vi "K_S30 Terminal-CN.vi"(8 "error in":errorcluster, 10 "request":u8[](array[numeric]), 11 "VISA resource":refnum<visa-resource-name>="COM2") -> (0 "error out":errorcluster, 2 "response":u8[](array[numeric]))   [LabVIEW 2022 SP3]
panel:
  out "msg and CRC":u8[](array[numeric])
  out "delited":u8[](array[numeric])
  # "Terminal for KELLER Transmitters Series3x \nV1.0, b.v.\n\nConfigure ComPort: use K_S30 OpenComPort --> Global Variable\n\nsend a message with CRC16 checksum, receive the reponse\ncheck CRC16, and exceptions\n\nerrors:\n0: no error\n1,2,3,32: exceptions thrown by the device: see comm. protocol\n100: broadcast\n-2: wrong echo from the RS485 converter\n-4: timeout\n-5: CRC16 wrong\nothers thrown by VISA"
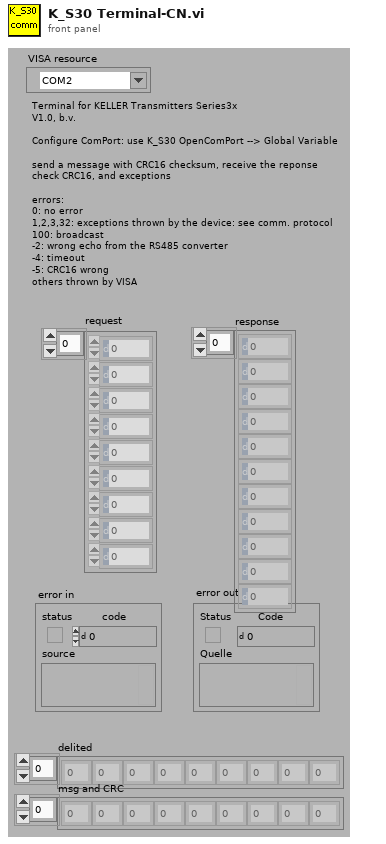
[diagram p1: front panel]
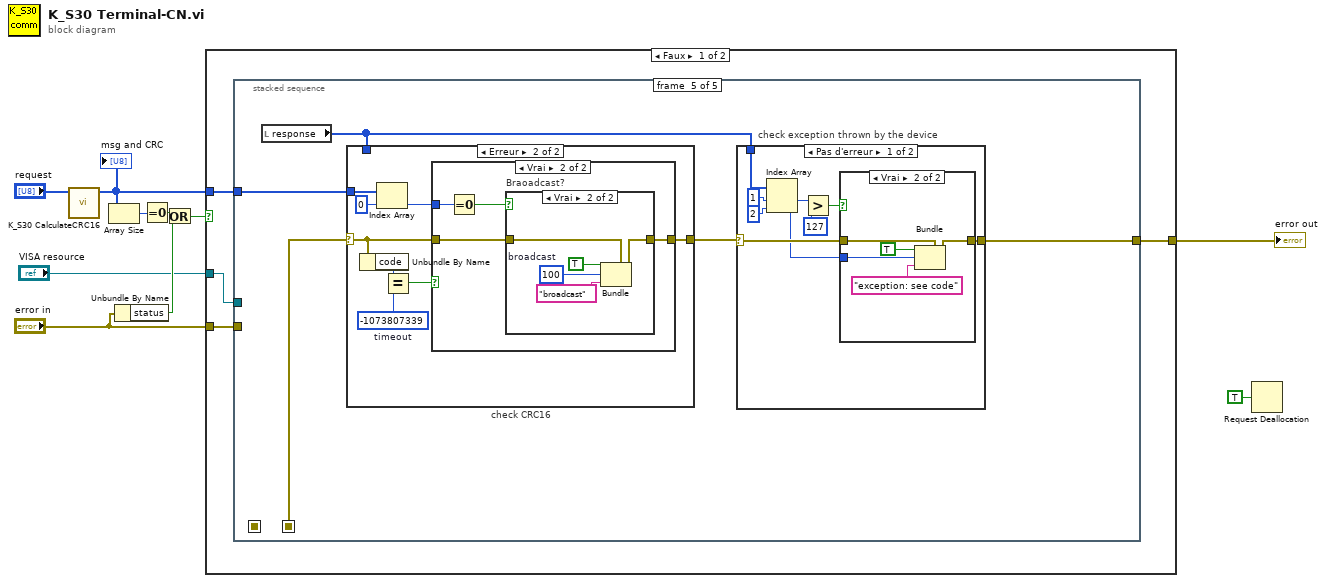
[diagram p0: block diagram]
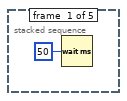
[diagram p2: hidden frame]
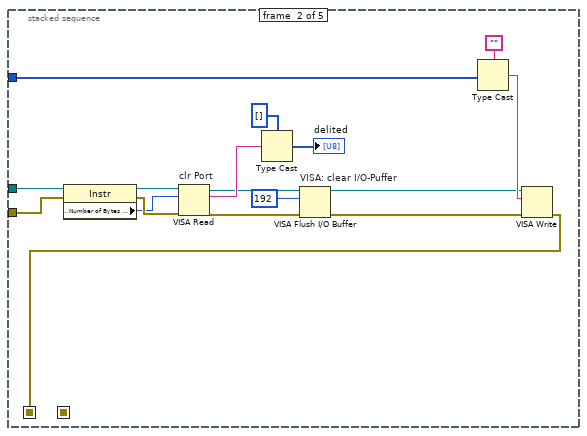
[diagram p3: hidden frame]
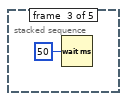
[diagram p4: hidden frame]
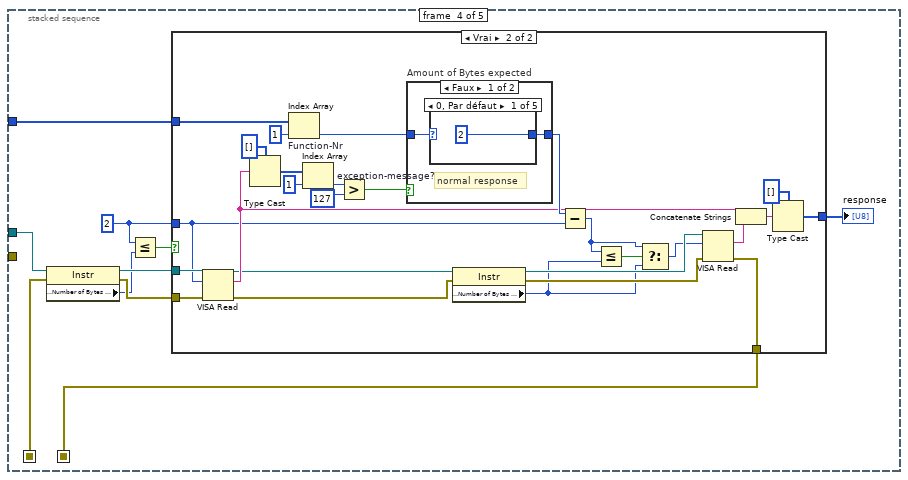
[diagram p5: hidden frame]
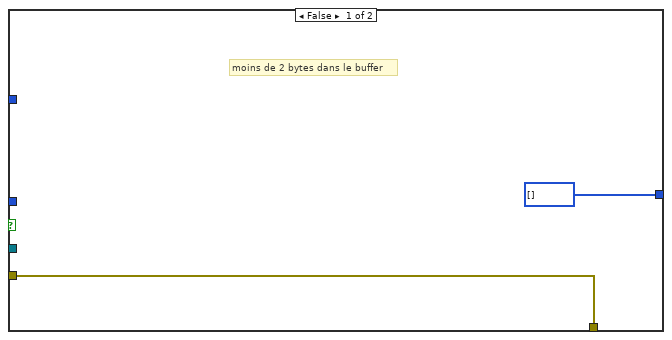
[diagram p6: hidden frame]
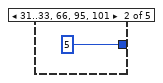
[diagram p7: hidden frame]
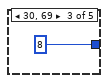
[diagram p8: hidden frame]
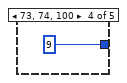
[diagram p9: hidden frame]
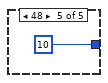
[diagram p10: hidden frame]
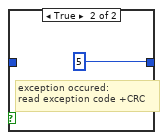
[diagram p11: hidden frame]
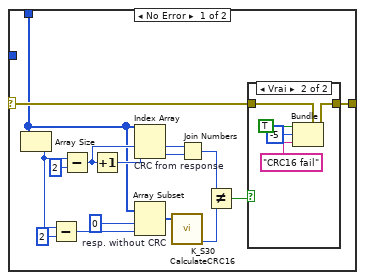
[diagram p14: hidden frame]
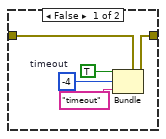
[diagram p17: hidden frame]
diagram:
  n1 = call "K_S30 CalculateCRC16.vi"("msg without CRC"="request") -> ("msg and CRC"=w4:u8[])  [unwired: 3 in, 3 out]
  "msg and CRC" <- w4
  n2 = Array Size(array=w4) -> (size(s)=w5:i32)
  n3 = Unbundle By Name("error in") -> ("status"=w7:bool)
  n4 = Equal To 0?(x=w5) -> (x = 0?=w8:bool)
  n5 = Or(x=w8, y=w7) -> (x .or. y?=w6:bool)
  n6 = case shown="Faux" w6 {
    tunnel: "VISA resource" -> [w14 _]
    tunnel: "error in" -> [w13 w147]
    tunnel: w4 -> [w12 _]
    tunnel: [w11 w147] -> w3
    frame False {
      n7 = stacked-sequence {
        seq-local: [_ w16 _ _ _] -> [_ _ _ w39 _]
        seq-local: [_ _ _ w41 _] -> [_ _ _ _ w82]
        tunnel: w14 -> [_ w28 _ w40 _]
        tunnel: w13 -> [_ w27 _ _ _]
        tunnel: w12 -> [_ w17 _ w43 w81]
        tunnel: [_ _ _ _ w83] -> w11
        frame #0 {
          n8 = Wait (ms)(milliseconds to wait=u32 50 ("ms Wartezeit")) -> ()  [unwired: 1 out]
        }
        frame #1 {
          n9 = property class="Instr"(reference=w28, error in=w27) -> (reference out=w32:refnum<visa-resource-name>, error out=w31:errorcluster, "Serial Settings:Number of Bytes at Serial Port"=w30:u32)
          n10 = VISA Read "clr Port"(VISA resource name=w32, byte count=w30, error in (no error)=w31) -> (VISA resource name out=w23:refnum<visa-resource-name>, read buffer=w26:string, error out=w24:errorcluster)  [unwired: 1 out]
          n11 = Type Cast(type=u8[] [], x=w26) -> (*(type *) &x=→"delited":u8[])
          n12 = VISA Flush I/O Buffer "VISA: clear I/O-Puffer"(VISA resource name=w23, mask (16)=u16 192 ("Maskieren (16)"), error in (no error)=w24) -> (VISA resource name out=w19:refnum<visa-resource-name>, error out=w18:errorcluster)
          n13 = Type Cast(type="", x=w17) -> (*(type *) &x=w20:string)
          n14 = VISA Write(VISA resource name=w19, write buffer=w20, error in (no error)=w18) -> (error out=w16:errorcluster)  [unwired: 2 out]
        }
        frame #2 {
          n15 = Wait (ms)(milliseconds to wait=u32 50 ("ms Wartezeit")) -> ()  [unwired: 1 out]
        }
        frame #3 {
          w36 = u32 2 ("Anzahl der Bytes (0)")
          n16 = property class="Instr"(reference=w40, error in=w39) -> (reference out=w38:refnum<visa-resource-name>, error out=w37:errorcluster, "Serial Settings:Number of Bytes at Serial Port"=w35:u32)
          n17 = Less Or Equal?(x=w36, y=w35) -> (x <= y?=w34:bool)
          n18 = case shown="Vrai" w34 {
            tunnel: w43 -> [_ w65]
            tunnel: [u8[] [] w58] -> w42
            tunnel: [w44 w57] -> w41
            tunnel: w38 -> [_ w56]
            tunnel: w37 -> [w44 w55]
            tunnel: w36 -> [_ w54]
            frame False {
              # "moins de 2 bytes dans le buffer"
            }
            frame True {
              n19 = VISA Read(VISA resource name=w56, byte count=w54, error in (no error)=w55) -> (VISA resource name out=w53:refnum<visa-resource-name>, read buffer=w61:string, error out=w52:errorcluster)  [unwired: 1 out]
              n20 = Type Cast(type=u8[] [], x=w61) -> (*(type *) &x=w71:u8[])
              n21 = Index Array "Function-Nr"(array=w65, index=1 ("Index")) -> (element=w64:u8)
              n22 = Index Array "exception-message?"(array=w71, index=1 ("Index")) -> (element=w69:u8)
              n23 = Greater?(x=w69, y=u8 127) -> (0:w67:bool)
              n24 = case "Amount of Bytes expected" shown="Faux" w67 {
                tunnel: w64 -> [w74 _]
                tunnel: [w73 u32 5] -> w63
                frame False {
                  # "normal response"
                  n25 = case shown="0, Par défaut" w74 {
                    tunnel: [u32 2 u32 5 u32 8 u32 9 u32 10] -> w73
                    frame 0, Default {
                    }
                    frame 31..33, 66, 95, 101 {
                    }
                    frame 30, 69 {
                    }
                    frame 73, 74, 100 {
                    }
                    frame 48 {
                    }
                  }
                }
                frame True {
                  # "exception occured:\nread exception code +CRC"
                }
              }
              n26 = property class="Instr"(reference=w53, error in=w52) -> (reference out=w51:refnum<visa-resource-name>, error out=w50:errorcluster, "Serial Settings:Number of Bytes at Serial Port"=w46:u32)
              n27 = Subtract(x=w63, y=w54) -> (x-y=w48:u32)
              n28 = Less Or Equal?(x=w48, y=w46) -> (x <= y?=w49:bool)
              n29 = Select(t=w48, s=w49, f=w46) -> (s? t:f=w47:u32)
              n30 = VISA Read(VISA resource name=w51, byte count=w47, error in (no error)=w50) -> (read buffer=w62:string, error out=w57:errorcluster)  [unwired: 2 out]
              n31 = Concatenate Strings(w61, w62) -> (w59:string)
              n32 = Type Cast(type=u8[] [], x=w59) -> (*(type *) &x=w58:u8[])
            }
          }
          "response" <- w42
        }
        frame #4 {
          n33 = local read "response"() -> (w84:u8[])
          n34 = case "check CRC16" shown="Erreur" w82 {
            selector: w82 -> [w104 w128]
            tunnel: [w103 w127] -> w85
            tunnel: w84 -> [w102 _]
            tunnel: w81 -> [_ w124]
            frame No Error {
              n35 = Array Size(array=w102) -> (size(s)=w116:i32)
              n36 = Subtract(x=w116, y=2) -> (x-y=w114:i32)
              n37 = Subtract(x=w116, y=2) -> (x-y=w110:i32)
              n38 = Increment(x=w110) -> (x+1=w111:i32)
              n39 = Index Array "CRC from response"(array=w102, index #1=w110, index #2=w111) -> (element #1=w109:u8, element #2=w108:u8)
              n40 = Array Subset "resp. without CRC"(array=w102, index=0 ("Index"), length=w114) -> (w112:u8[])
              n41 = call "K_S30 CalculateCRC16.vi"("msg without CRC"=w112) -> ("CRC16"=w106:u16)  [unwired: 3 in, 3 out]
              n42 = Join Numbers(hi=w109, lo=w108) -> ((hi.lo)=w107:u16)
              n43 = Not Equal?(x=w107, y=w106) -> (x != y?=w105:bool)
              n44 = case shown="Vrai" w105 {
                tunnel: w104 -> [w118 w123]
                tunnel: [w118 w119] -> w103
                frame False {
                }
                frame True {
                  n45 = Bundle(cluster=w123, "status"=TRUE, "code"=-5, "source"="CRC16 fail") -> (w119:errorcluster)
                }
              }
            }
            frame Error {
              w130 = -1073807339  # timeout
              n46 = Unbundle By Name(w128) -> ("code"=w131:i32)
              n47 = Index Array(array=w124, index=0 ("Index")) -> (element=w125:u8)
              n48 = Equal?(x=w131, y=w130) -> (x = y?=w129:bool)
              n49 = case shown="Vrai" w129 {
                tunnel: w128 -> [w132 w136]
                tunnel: [w132 w135] -> w127
                tunnel: w125 -> [_ w134]
                frame False {
                }
                frame True {
                  n50 = Equal To 0?(x=w134) -> (x = 0?=w133:bool)
                  n51 = case "Braoadcast?" shown="Vrai" w133 {
                    tunnel: w136 -> [w139 w143]
                    tunnel: [w138 w142] -> w135
                    frame False {
                      w137 = -4  # timeout
                      n52 = Bundle(cluster=w139, "status"=TRUE, "code"=w137, "source"="timeout") -> (w138:errorcluster)
                    }
                    frame True {
                      w144 = 100  # broadcast
                      n53 = Bundle(cluster=w143, "status"=TRUE, "code"=w144, "source"="broadcast") -> (w142:errorcluster)
                    }
                  }
                }
              }
            }
          }
          n54 = case "check exception thrown by the device" shown="Pas d'erreur" w85 {
            selector: w85 -> [w89 w101]
            tunnel: [w88 w101] -> w83
            tunnel: w84 -> [w91 _]
            frame No Error {
              n55 = Index Array(array=w91, index #1=1 ("Index"), index #2=2 ("Index")) -> (element #1=w93:u8, element #2=w86:u8)
              n56 = Greater?(x=w93, y=u8 127) -> (0:w90:bool)
              n57 = case shown="Vrai" w90 {
                tunnel: w89 -> [w95 w98]
                tunnel: [w95 w97] -> w88
                tunnel: w86 -> [_ w96]
                frame False {
                }
                frame True {
                  n58 = Bundle(cluster=w98, "status"=TRUE, "code"=w96, "source"="exception: see code") -> (w97:errorcluster)
                }
              }
            }
            frame Error {
            }
          }
        }
      }
    }
    frame True {
    }
  }
  "error out" <- w3
  n59 = Request Deallocation(TRUE ("flag")) -> ()
